vi "Lire prog MODBUS EPC.vi"(3 "error in (no error)":errorcluster caption="entrée d'erreur (pas d'erreur)", 4 "Numéro de programme":u8, 5 "Adresse rég":u8 caption="Adresse régulateur", 6 "Port COM run 1 REG":refnum<visa-resource-name>) -> (0 "error out":errorcluster caption="entrée d'erreur (pas d'erreur)", 1 "annulé":bool, 2 "Programme":T1(array[cluster]))   [LabVIEW 2022 SP3]
uses:
  Enum/Enum r6.ctl
panel:
  out "erreur seg":errorcluster caption="erreur par segment"
  in  "Annuler":bool
  out "données générales":u16[](array[numeric])
  out "Nom rég":string caption="Nom régulateur"
  out "No seg":u8 caption="Numéro du segment"
  # "lecture profil"
  # "unités rampe"
  # "unités palier"
  # "nb cycles"
  # "type fin"
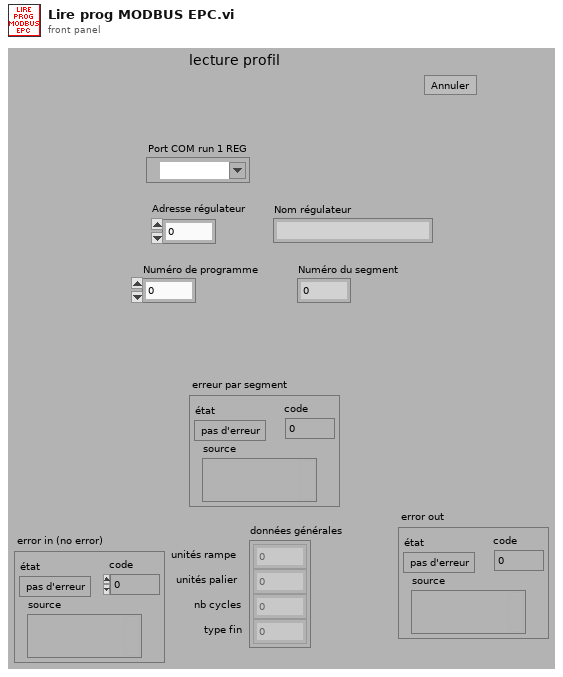
[diagram p1: front panel]
types:
  T1 = cluster{"chaîne o":string, "Received Value":dbl}[][]
  T2 = typedef "Enum r6.ctl" = enum16{"sélection programme", "données générales", "segments", "fin de prog", "fin"}
  T3 = cluster{"chaîne o":string, "Received Value":dbl}[]
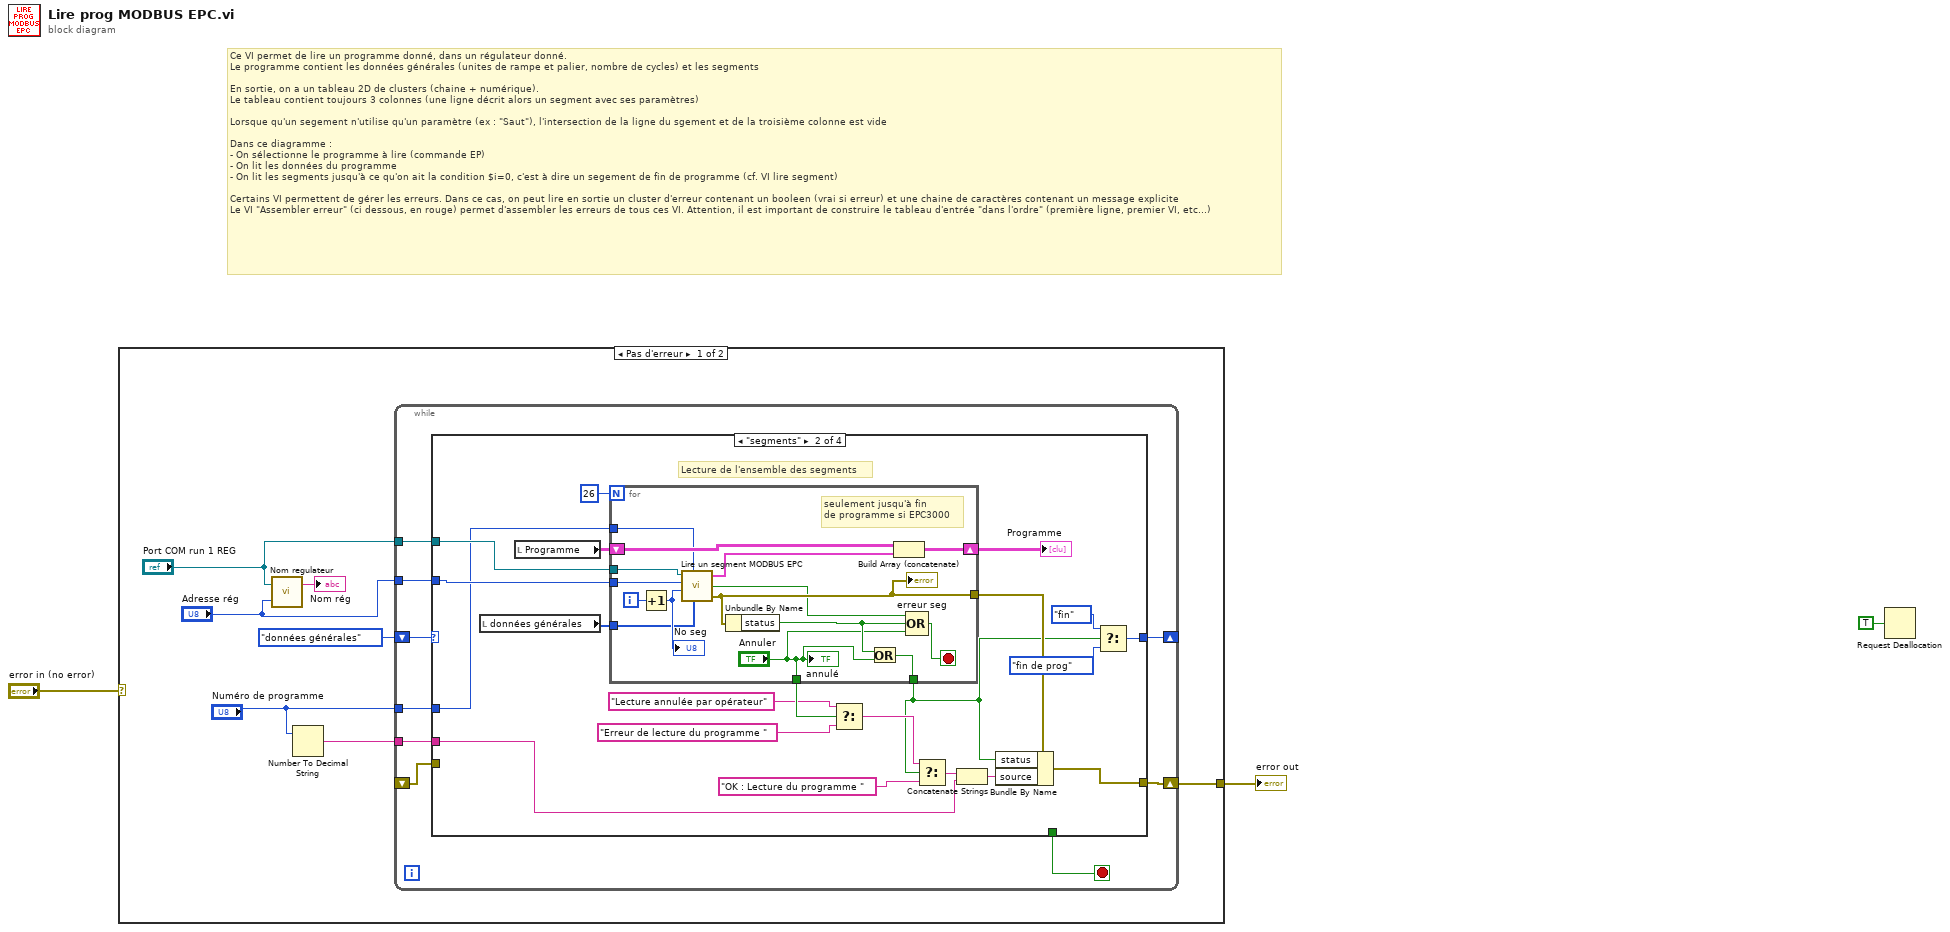
[diagram p0: block diagram]
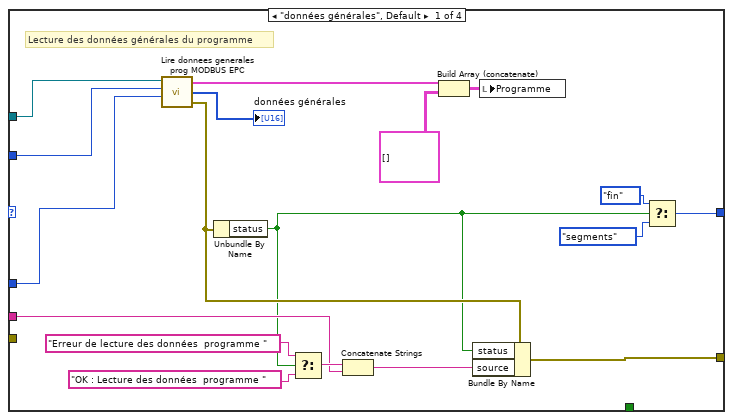
[diagram p2: hidden frame]
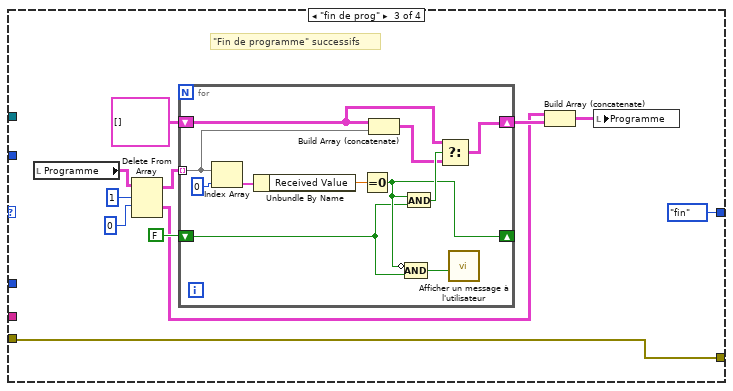
[diagram p3: hidden frame]
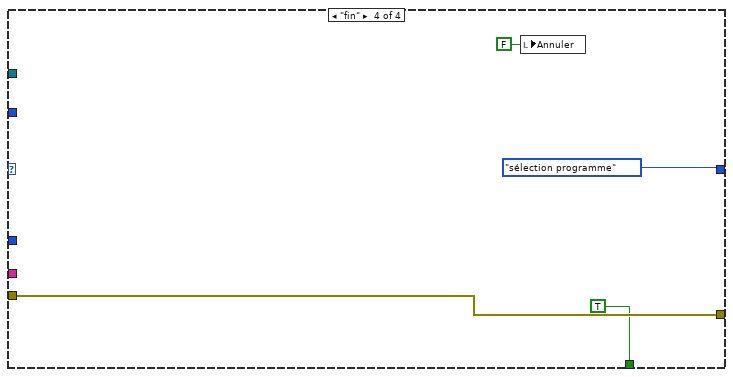
[diagram p4: hidden frame]
diagram:
  # "Ce VI permet de lire un programme donné, dans un régulateur donné.\nLe programme contient les données générales (unites de rampe et palier, nombre de cycles) et les segments\n\nEn sortie, on a un tableau 2D de clusters (chaine + numérique). \nLe tableau contient toujours 3 colonnes (une ligne décrit alors un segment avec ses paramètres)\n\nLorsque qu'un segement n'utilise qu'un paramètre (ex : \"Saut\"), l'intersection de la ligne du sgement et de la troisième colonne est vide\n\nDans ce diagramme : \n- On sélectionne le programme à lire (commande EP)\n- On lit les données du programme\n- On lit les segments jusqu'à ce qu'on ait la condition $i=0, c'est à dire un segement de fin de programme (cf. VI lire segment)\n\nCertains VI permettent de gérer les erreurs. Dans ce cas, on peut lire en sortie un cluster d'erreur contenant un booleen (vrai si erreur) et une chaine de caractères contenant un message explicite\nLe VI \"Assembler erreur\" (ci dessous, en rouge) permet d'assembler les erreurs de tous ces VI. Attention, il est important de construire le tableau d'entrée \"dans l'ordre\" (première ligne, premier VI, etc...)"
  n1 = case shown="Pas d'erreur" "error in (no error)" {
    selector: "error in (no error)" -> [_ w100]
    tunnel: [w4 w100] -> w2
    frame No Error {
      n2 = call "Nom regulateur.vi"("Adresse régulateur"="Adresse rég", "Port COM run 1 REG"="Port COM run 1 REG") -> ("Nom régulateur"=→"Nom rég":string)  [unwired: 1 in]
      n3 = Number To Decimal String(number="Numéro de programme") -> (decimal integer string=w7:string)  [unwired: 1 in]
      n4 = while {
        shift-right: [w13] -> _
        shift-left: Enum_r6."données générales" ("Énum") -> [w19]
        tunnel: "Port COM run 1 REG" -> [w18]
        tunnel: "Adresse rég" -> [w17]
        tunnel: "Numéro de programme" -> [w16]
        tunnel: w7 -> [w15]
        shift-right: [w14] -> w4
        shift-left: _ -> [w12]
        stop <- w11 stop-if-true
        n5 = case shown="\"segments\"" w19 {
          tunnel: w18 -> [w32 w53 _ _]
          tunnel: w17 -> [w31 w52 _ _]
          tunnel: w16 -> [w21 w45 _ _]
          tunnel: w15 -> [w29 w51 _ _]
          tunnel: [w30 w50 w83 w99] -> w14
          tunnel: [w22 w47 Enum_r6."fin" ("Énum") Enum_r6."sélection programme" ("Énum")] -> w13
          tunnel: w12 -> [_ _ w83 w99]
          tunnel: [_ _ _ TRUE] -> w11
          frame "données générales", Default {
            # "Lecture des données générales du programme"
            n6 = call "Lire donnees generales prog MODBUS EPC.vi"("N° prog"=w21, "Adresse régulateur"=w31, "Port COM"=w32) -> ("error out"=w37:errorcluster, "données générales"=→"données générales":u16[], "Programmation données"=w27:cluster{"chaîne o":string, dbl}[])  [unwired: 1 in]
            n7 = Unbundle By Name(w37) -> ("status"=w25:bool)
            n8 = Select(t="Erreur de lecture des données  programme ", s=w25, f="OK : Lecture des données  programme ") -> (s? t:f=w34:string)
            n9 = Concatenate Strings(w34, w29) -> (w33:string)
            n10 = Build Array (concatenate)(w27, T1 []) -> (w26:T1)
            n11 = Bundle By Name(cluster=w37, "status"=w25, "source"=w33) -> (w30:errorcluster)
            n12 = local write "Programme"(w26) -> ()
            n13 = Select(t=Enum_r6."fin" ("Énum"), s=w25, f=Enum_r6."segments" ("Énum")) -> (s? t:f=w22:T2)
          }
          frame "segments" {
            # "Lecture de l'ensemble des segments"
            n14 = local read "données générales"() -> (w44:u16[])
            n15 = local read "Programme"() -> (w54:T1)
            n16 = for {
              N: 26 -> [_]
              tunnel: w52 -> [w73]
              shift-right: [w68] -> w46
              shift-left: w54 -> [w72]
              tunnel: [w65] -> w58
              tunnel: w53 -> [w69]
              tunnel: w45 -> [w66]
              tunnel: w44 -> [w64]
              tunnel: ["Annuler"] -> w43
              tunnel: [w60] -> w39
              i -> [w71]
              stop <- w63 stop-if-true
              # "seulement jusqu'à fin\nde programme si EPC3000"
              n17 = Increment(x=w71) -> (x+1=w67:i32)
              "No seg" <- w67
              n18 = call "Lire un segment MODBUS EPC.vi"("Port COM"=w69, "No prog"=w66, "Adresse régulateur"=w73, "Numéro de segment"=w67, "données générales"=w64) -> ("Programmation Segment"=w70:T3, "Fin de programme"=w59:bool, "error out"=w65:errorcluster)  [unwired: 1 in]
              "erreur seg" <- w65
              n19 = Unbundle By Name(w65) -> ("status"=w62:bool)
              n20 = Or(x=w62, y="Annuler") -> (x .or. y?=w60:bool)
              n21 = Build Array (concatenate)(w72, w70) -> (w68:T1)
              n22 = Compound Arithmetic op=OR ("Opérateur arithmétique")(w59, w62, "Annuler") -> (w63:bool)
              "annulé" <- "Annuler"
            }
            "Programme" <- w46
            n23 = Select(t="Lecture annulée par opérateur", s=w43, f="Erreur de lecture du programme ") -> (s? t:f=w40:string)
            n24 = Select(t=w40, s=w39, f="OK : Lecture du programme ") -> (s? t:f=w57:string)
            n25 = Concatenate Strings(w57, w51) -> (w56:string)
            n26 = Bundle By Name(cluster=w58, "status"=w39, "source"=w56) -> (w50:errorcluster)
            n27 = Select(t=Enum_r6."fin" ("Énum"), s=w39, f=Enum_r6."fin de prog" ("Énum")) -> (s? t:f=w47:T2)
          }
          frame "fin de prog" {
            # "\"Fin de programme\" successifs"
            n28 = local read "Programme"() -> (w80:T1)
            n29 = Delete From Array(array=w80, length=1 ("longueur"), index (row)=0 ("indice (ligne)")) -> (deleted portion=w74:T1, array with subset deleted=w76:T1)  [unwired: 1 in]
            n30 = for {
              tunnel: w76 -> [w92] mode=indexing
              shift-right: [w87] -> _
              shift-left: FALSE -> [w86]
              shift-right: [w89] -> w78
              shift-left: T1 [] -> [w88]
              n31 = Index Array(array=w92, index=0 ("indice")) -> (element=w94:cluster{"chaîne o":string, "Received Value":dbl})
              n32 = Unbundle By Name(w94) -> ("Received Value"=w93:dbl)
              n33 = Equal To 0?(x=w93) -> (x = 0?=w87:bool)
              n34 = Build Array (concatenate)(w88, w92) -> (w90:T1)
              n35 = And(x=w87, y=w86) -> (x .and. y?=w91:bool)
              n36 = Compound Arithmetic op=AND ("Opérateur arithmétique")(invert w87, w86) -> (w85:bool)
              n37 = Select(t=w88, s=w91, f=w90) -> (s? t:f=w89:T1)
              n38 = call "Afficher un message à l'utilisateur"("Enable"=w85) -> ()  [unwired: 9 in, 2 out]
            }
            n39 = Build Array (concatenate)(w74, w78) -> (w77:T1)
            n40 = local write "Programme"(w77) -> ()
          }
          frame "fin" {
            n41 = local write "Annuler"(FALSE ("Annuler")) -> ()
          }
        }
      }
    }
    frame Error {
    }
  }
  "error out" <- w2
  n42 = Request Deallocation(TRUE ("flag")) -> ()
